vi "09_another_example.vi"() -> ()   [LabVIEW 2018, in "LV2Julia_examples.lvlib"]
uses:
  LV2Julia_examples.lvlib
  LV2Julia_core/VIs/Server or client state.ctl
  LV2Julia_core/VIs/detailed error info.ctl
  LV2Julia_core/VIs/StackFrame.ctl
  simple examples functions.ctl
  LV2Julia_core/VIs/Commands.ctl
  63b50369-e720-4ad2-b7fe-b63add1d9180.vi
  edf81fa3-46bf-427f-9605-85b461656974.vi
  29886417-d43f-41fb-9c0c-469db3f8c96d.vi
  3fe35f36-217a-40a5-a789-8326c52a1f5c.vi
  8d86b089-302c-401c-ae82-d9ebdf0ff266.vi
  35a44a82-786b-41ea-be73-9a4468e4df9d.vi
  a43e0667-dcfc-466a-94c9-f7da2d4fd36f.vi
  <vilib>/Utility/High Resolution Relative Seconds.vi
  edf81fa3-46bf-427f-9605-85b461656974.vi/5942f0bd-7063-4fdb-8e1f-163338074038.vi
  29886417-d43f-41fb-9c0c-469db3f8c96d.vi/94a9aba0-1697-4c84-91eb-fcc68cde7b35.vi
  3fe35f36-217a-40a5-a789-8326c52a1f5c.vi/ea1c78d1-8dec-492d-b19c-ac119526c4b9.vi
  35a44a82-786b-41ea-be73-9a4468e4df9d.vi/a5fe95ae-8dc8-4e69-84a5-09934be0e8db.vi
  35a44a82-786b-41ea-be73-9a4468e4df9d.vi/54b1eeee-b135-46c6-a027-240f26ec244c.vi
  35a44a82-786b-41ea-be73-9a4468e4df9d.vi/29dc6209-e462-4798-844e-48d2ff1efa69.vi
  35a44a82-786b-41ea-be73-9a4468e4df9d.vi/fb13ef7b-3dc2-43ae-b026-48829507478f.vi
  edf81fa3-46bf-427f-9605-85b461656974.vi/5942f0bd-7063-4fdb-8e1f-163338074038.vi/a212b533-a802-43cc-9280-c521d8aa8d2c.vi
  29886417-d43f-41fb-9c0c-469db3f8c96d.vi/94a9aba0-1697-4c84-91eb-fcc68cde7b35.vi/986b3ef1-05af-4579-a01d-89cf0a7e1e70.vi
  29886417-d43f-41fb-9c0c-469db3f8c96d.vi/94a9aba0-1697-4c84-91eb-fcc68cde7b35.vi/f2b0486c-a7c3-4e7a-a904-fec8be3410f0.vi
  29886417-d43f-41fb-9c0c-469db3f8c96d.vi/94a9aba0-1697-4c84-91eb-fcc68cde7b35.vi/dd0e1e63-28cb-45cd-b055-498631b7826e.vi
  3fe35f36-217a-40a5-a789-8326c52a1f5c.vi/ea1c78d1-8dec-492d-b19c-ac119526c4b9.vi/ce52c93b-e6e4-494b-9f4d-7b7b02eec5ed.vi
  3fe35f36-217a-40a5-a789-8326c52a1f5c.vi/ea1c78d1-8dec-492d-b19c-ac119526c4b9.vi/7b140ace-ff7d-49f7-89b3-e9a714b2692c.vi
  3fe35f36-217a-40a5-a789-8326c52a1f5c.vi/ea1c78d1-8dec-492d-b19c-ac119526c4b9.vi/f14f8910-dfb7-4812-9577-bccbd49d3442.vi
  35a44a82-786b-41ea-be73-9a4468e4df9d.vi/a5fe95ae-8dc8-4e69-84a5-09934be0e8db.vi/43619f87-d3a3-4430-b781-19a1ed80452b.vi
  35a44a82-786b-41ea-be73-9a4468e4df9d.vi/a5fe95ae-8dc8-4e69-84a5-09934be0e8db.vi/6bcf3c00-a23e-49d9-b22d-a7ee64d807ae.vi
  edf81fa3-46bf-427f-9605-85b461656974.vi/5942f0bd-7063-4fdb-8e1f-163338074038.vi/a212b533-a802-43cc-9280-c521d8aa8d2c.vi/2d6b78cf-7cb1-4e49-bbcd-7392787414f6.vi
  35a44a82-786b-41ea-be73-9a4468e4df9d.vi/a5fe95ae-8dc8-4e69-84a5-09934be0e8db.vi/43619f87-d3a3-4430-b781-19a1ed80452b.vi/46c53f12-cc20-4ee9-bbe7-34102a510572.vi
  LV2Julia_core/VIs/jl-scripts path.vi
  LV2Julia_core/VIs/check ID validity.vi
  LV2Julia_core/VIs/bindata_descr to JSON.vi
  LV2Julia_core/VIs/check cluster field names.vi
  LV2Julia_core/VIs/concat JSON.vi
  LV2Julia_core/VIs/build request.vi
  LV2Julia_core/VIs/Parse server response.vi
  LV2Julia_core/VIs/log jl exceptions.vi
  <vilib>/Utility/error.llb/Error Cluster From Error Code.vi
  LV2Julia_core/LV2Julia_core.lvlib
  <vilib>/measure/NI_MABase.lvlib
panel:
  out "ZMQ timeout":bool
  out "Julia script file path":path
  out "temporary script path":path
  out "Jl Server state":T1
  in  "execution control pages":enum32{"Start", "go - test"}(tab)
  in  "go":bool caption="go (Julia Server started externally)"
  in  "Start with Julia":bool caption="Start Julia Server and go"
  in  "ZMQ endpoint":string="tcp://127.0.0.1:5555"
  in  "p":dbl=1.0
  in  "fn":T2 caption="select function at Server" items=["arr_amplitude", "arr_length", "arr_mean", "arr_median", "arr_rms", "vec_amplify", "vec_attenuate", "vec_power"]
  in  "trim @ begin":dbl min=0.0 max=100.0 step=1.0 format="%#.1f%%"
  in  "trim @ end":dbl min=0.0 max=200.0 step=1.0 format="%#.1f%%"
  in  "Group":T3(tab)
  out "Server response":dbl
  out "data received plot":dbl[](graph)
  out "data received":dbl[](array[numeric]) format="%.3f"
  out "RMS":dbl
  out "detailed error info":T4
  out "current error":errorcluster
  out "final error":errorcluster
  out "short err code":u8
  in  "tones":T6(array[cluster])=[{"frequency"=10.0, "amplitude"=1.0, "phase"=0.0}, {"frequency"=20.0, "amplitude"=0.1, "phase"=0.0}] {"phase" format="%.2p"; "amplitude" format="%0.2p"; "frequency" format="%0.2p"}
  in  "noise (rms)":dbl=0.1 format="%.2p"
  in  "offset":dbl format="%.2p"
  in  "sampling info":cluster{"Fs":dbl, "#s":dbl}={"Fs"=1000.0, "#s"=1000.0} {"Fs" format="%.2p"}
  in  "next":bool
  out "data sent to server":dbl[](graph)
  out "data sent":dbl[](array[numeric]) format="%.3f"
  out "function name":string
  in  "stop this VI only":bool
  in  "stop both this VI and Julia Server":bool
  out "call duration (ms)":dbl format="%#.2f"
  # "tcp://127.0.0.1:5555 \nfor local Julia Server\n\nFor a Julia Server running on a separate computer,  you probably must use an IPv4 address in numeric form (not a DNS name) - see https://stackoverflow.com/questions/6024003/why-doesnt-zeromq-work-on-localhost.\n\nThis control only used if Julia Server is not being started by this VI."
  # "generate sample array"
  # "function and parameter"
  # "enter a negative or a large positive value to cause an exception"
  # "data returned by server"
  # "data sent to server"
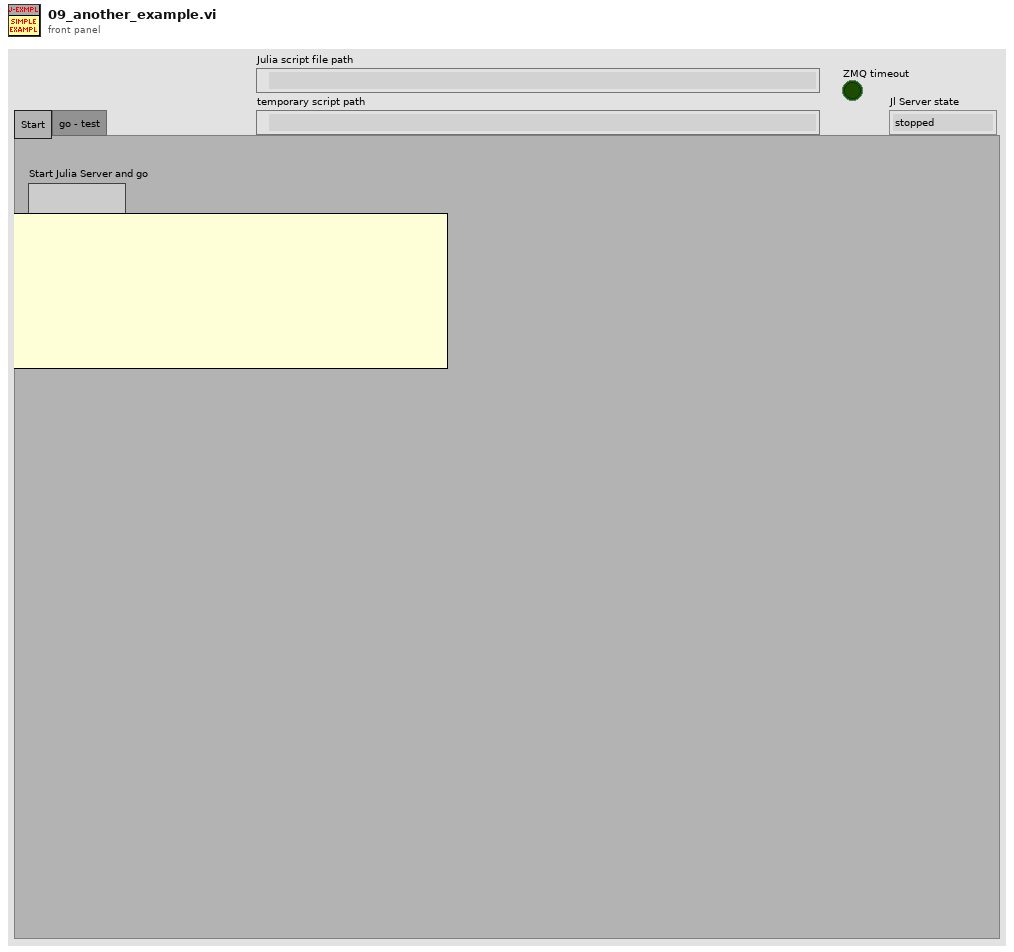
[diagram p1: front panel]
types:
  T1 = typedef "LV2Julia_core.lvlib/Server or client state.ctl" = enum16{"stopped", "running", "unknown"}
  T2 = typedef "LV2Julia_examples.lvlib/simple examples functions.ctl" = u16
  T3 = enum32{"fns returning scalar", "fns returning vector", "error"}
  T4 = typedef "LV2Julia_core.lvlib/detailed error info.ctl" = cluster{"exception_or_info":string, "trace":T5[]}
  T5 = typedef "LV2Julia_core.lvlib/StackFrame.ctl" = cluster{"frame_summary":string, "func":string, "linfo":string, "file":string, "line":i32, "pointer":u64, "from_c":bool, "inlined":bool}
  T6 = cluster{"frequency":dbl, "amplitude":dbl, "phase":dbl}[]
  T7 = typedef "LV2Julia_core.lvlib/Commands.ctl" = enum16{"Start Jl-server & Init LV-client", "Send request & Get response ", "Stop Jl-server & Cleanup LV-client", "Cleanup LV-client", "Start Jl-server", "Stop Jl-server", "Init LV-Client", "Cleanup LV-Client", "(not allowed)", "Set LV Client state", "Set Jl Server state", "set ZMQ timeout", "read ZMQ timeout", "read-out state"}
  T8 = enum8{"Enabled", "Disabled", "Disabled and Grayed Out"}
  T9 = typedef "LV2Julia_core.lvlib/Bindata&description.ctl" = cluster{"bindata_descr":T10[], "bindata":u8[]}
  T10 = typedef "LV2Julia_core.lvlib/Bindata description.ctl" = cluster{"nofbytes":i32, "numtype":string, "start":i32, "arrdims":i32[], "kwarg_name":string, "category":string}
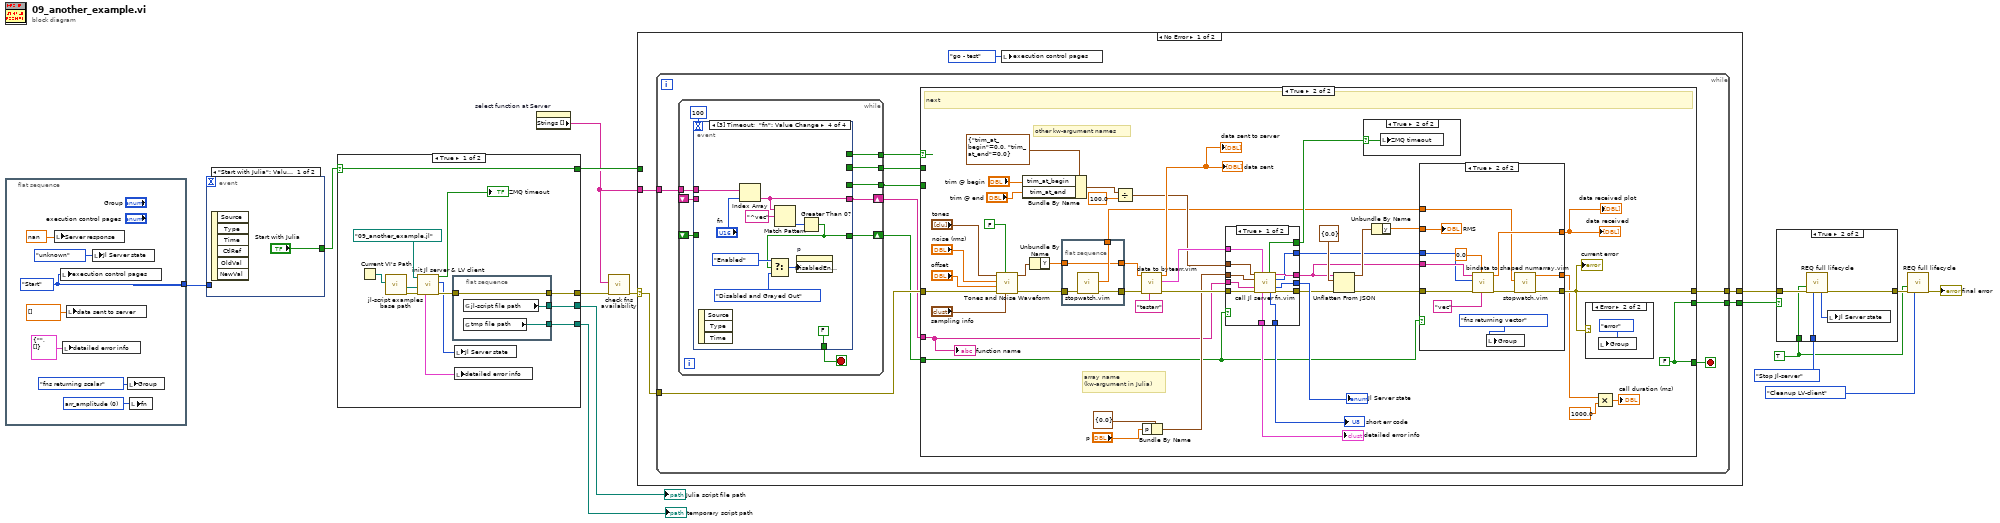
[diagram p0: block diagram]
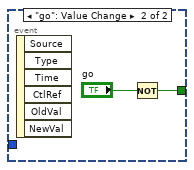
[diagram p2: hidden frame]
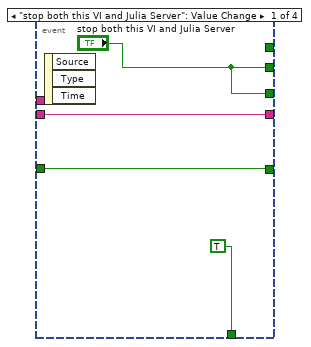
[diagram p3: hidden frame]
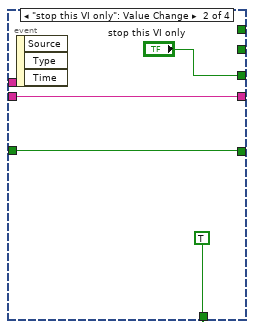
[diagram p4: hidden frame]
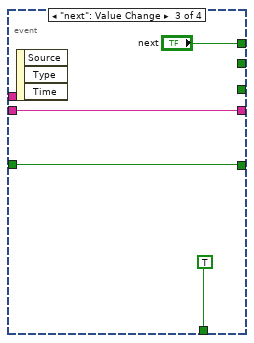
[diagram p5: hidden frame]
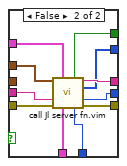
[diagram p7: hidden frame]
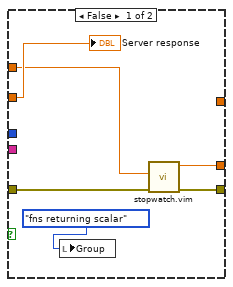
[diagram p9: hidden frame]
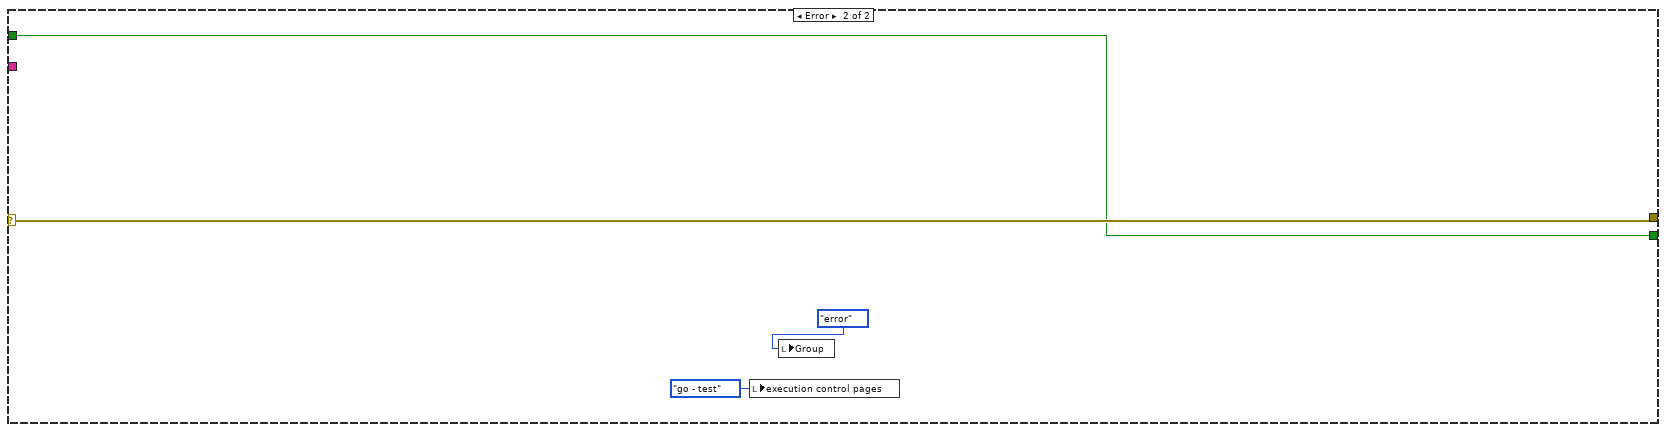
[diagram p11: hidden frame]
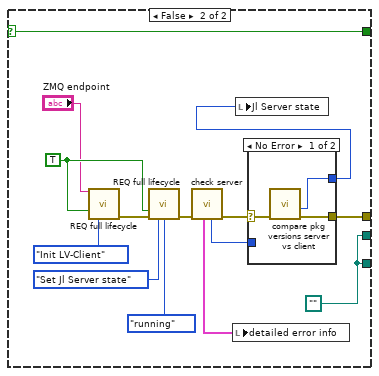
[diagram p12: hidden frame]
diagram:
  w10 = TRUE ("Force command")
  n1 = flat-sequence {
    tunnel: [w22] -> w6
    frame #0 {
      w16 = T2 0 items=["arr_amplitude", "arr_length", "arr_mean", "arr_median", "arr_rms", "vec_amplify", "vec_attenuate", "vec_power"] ("fn")
      w22 = enum32{"Start", "go - test", "finish"}."Start" ("execution control pages")
      n2 = local write "Server response"(nan ("Server response")) -> ()
      n3 = local write "execution control pages"(w22) -> ()
      n4 = local write "detailed error info"(T4 {"exception_or_info"="", "trace"=[]} ("detailed error info")) -> ()
      n5 = local write "data sent to server"(dbl[] []) -> ()
      n6 = local write "Jl Server state"(Server_or_client_state."unknown" ("Jl Server state out")) -> ()
      n7 = local write "Group"(T3."fns returning scalar" ("Group")) -> ()
      n8 = local write "fn"(w16) -> ()
    }
  }
  n9 = event shown="[0] \"Start with Julia\": Value Change" {
    selector: _ -> [_ _]
    dyn-events: _ -> [_ _]
    timeout: _ -> [_ _]
    tunnel: ["Start with Julia" w24] -> w8
    tunnel: w6 -> [_ _]
    event "Start with Julia": Value Change {
      n10 = event-data() -> ()  [unwired: 1 in, 6 out]
    }
    event "go": Value Change {
      n11 = event-data() -> ()  [unwired: 1 in, 6 out]
      n12 = Not(x="go") -> (.not. x?=w24:bool)
    }
  }
  n13 = case shown="True" w8 {
    selector: w8 -> [w37 w50]
    tunnel: [w36 w44] -> w5
    tunnel: [w37 w50] -> w7
    tunnel: [w35 w47] -> w1
    tunnel: [w34 w47] -> w2
    frame True {
      n14 = Current VI's Path() -> (path=w29:path)
      n15 = call "jl-script examples base path.vi"("calling example VI path"=w29) -> ("error out"=w28:errorcluster, "jl-script-examples base path"=w27:path)  [unwired: 9 in]
      n16 = call "init Jl server & LV client.vi"("error in (no error)"=w28, "Base path (not a path)"=w27, "Julia user functions script"=path "09_another_example.jl") -> ("error out"=w31:errorcluster, "Jl Server state out"=w30:T1, "timeout?"=→"ZMQ timeout":bool, "detailed error info"=w26:T4)  [unwired: 3 in, 2 out]
      n17 = flat-sequence {
        tunnel: [w40] -> w36
        tunnel: w31 -> [w40]
        tunnel: [w39] -> w35
        tunnel: [w38] -> w34
        frame #0 {
          n18 = global read "jl-scripts path.vi" "jl-script file path"() -> (w39:path)
          n19 = global read "jl-scripts path.vi" "tmp file path"() -> (w38:path)
        }
      }
      n20 = local write "Jl Server state"(w30) -> ()
      n21 = local write "detailed error info"(w26) -> ()
    }
    frame False {
      w47 = path ""
      w52 = TRUE ("Force command")
      n22 = call "REQ full lifecycle.vi"("ZMQ endpoint"="ZMQ endpoint", "Force command"=w52, "command"=Commands."Init LV-Client") -> ("error out"=w49:errorcluster)  [unwired: 6 in, 6 out]
      n23 = call "REQ full lifecycle.vi"("Force command"=w52, "error in"=w49, "command"=Commands."Set Jl Server state", "Jl Server state in"=Server_or_client_state."running") -> ("error out"=w48:errorcluster)  [unwired: 5 in, 6 out]
      n24 = call "check server.vi"("error in"=w48) -> ("error out"=w45:errorcluster, "Jl Server state out"=w43:T1, "detailed error info"=w41:T4)  [unwired: 6 in, 2 out]
      n25 = local write "detailed error info"(w41) -> ()
      n26 = case shown="No Error" w45 {
        selector: w45 -> [w57 w59]
        tunnel: [w56 w59] -> w44
        tunnel: [w55 w58] -> w42
        tunnel: w43 -> [_ w58]
        frame No Error {
          n27 = call "compare pkg versions server vs client.vi"("error in (no error)"=w57) -> ("error out"=w56:errorcluster, "Jl Server state out"=w55:T1)  [unwired: 5 in, 4 out]
        }
        frame Error {
        }
      }
      n28 = local write "Jl Server state"(w42) -> ()
    }
  }
  "temporary script path" <- w2
  "Julia script file path" <- w1
  n29 = property on="select function at Server" class="Ring (strict)"() -> ("Strings []"=w3:string[])  [unwired: 2 in, 2 out]
  n30 = call "check fns availability.vi"("error in (no error)"=w5, "fns list is"=w3) -> ("error out"=w4:errorcluster)  [unwired: 3 in, 6 out]
  n31 = case shown="No Error" w4 {
    selector: w4 -> [w63 w204]
    tunnel: [w64 w204] -> w15
    tunnel: [w62 w203] -> w9
    tunnel: w3 -> [w61 _]
    tunnel: w7 -> [_ w203]
    frame No Error {
      n32 = while {
        tunnel: w63 -> [w73]
        tunnel: [w74] -> w64
        tunnel: [w70] -> w62
        tunnel: w61 -> [w68]
        stop <- w71 stop-if-true
        n33 = while {
          tunnel: [w84] -> w72
          tunnel: [w83] -> w69
          tunnel: w68 -> [w80]
          shift-right: [w79] -> w67
          shift-left: _ -> [w76]
          shift-right: [w78] -> w66
          shift-left: _ -> [w77]
          tunnel: [w75] -> w65
          stop <- w82 stop-if-true
          n34 = event shown="[3] Timeout;  \"fn\": Value Change" {
            selector: _ -> [_ _ _ _]
            dyn-events: _ -> [_ _ _ _]
            timeout: 100 -> [_ _ _ _]
            tunnel: ["stop both this VI and Julia Server" _ _ _] -> w83
            tunnel: [_ _ "next" _] -> w84
            tunnel: [TRUE TRUE TRUE FALSE] -> w82
            tunnel: w80 -> [_ _ _ w100]
            tunnel: [w86 w90 w94 w99] -> w79
            tunnel: [w87 w91 w93 w98] -> w78
            tunnel: w77 -> [w87 w91 w93 _]
            tunnel: w76 -> [w86 w90 w94 _]
            tunnel: ["stop both this VI and Julia Server" "stop this VI only" _ _] -> w75
            event "stop both this VI and Julia Server": Value Change {
              n35 = event-data() -> ()  [unwired: 1 in, 3 out]
            }
            event "stop this VI only": Value Change {
              n36 = event-data() -> ()  [unwired: 1 in, 3 out]
            }
            event "next": Value Change {
              n37 = event-data() -> ()  [unwired: 1 in, 3 out]
            }
            event Timeout; Value Change {
              n38 = event-data() -> ()  [unwired: 1 in, 3 out]
              n39 = Index Array(array=w100, index="fn") -> (element=w98:string)
              n40 = Match Pattern(string=w98, regular expression="^vec") -> (offset past match=w104:i32)  [unwired: 1 in, 3 out]
              n41 = Greater Than 0?(x=w104) -> (x > 0?=w99:bool)
              n42 = Select(t=T8."Enabled" ("Disabled"), s=w99, f=T8."Disabled and Grayed Out" ("Disabled")) -> (s? t:f=w106:T8)
              n43 = property on="p" class="DigNum (strict)"("DisabledEnum"=w106) -> ()  [unwired: 2 in, 2 out]
            }
          }
        }
        n44 = case shown="True" w72 {
          tunnel: [w109 w136] -> w74
          tunnel: w73 -> [w109 w141]
          tunnel: [w108 w140] -> w71
          tunnel: w65 -> [w108 _]
          tunnel: [w107 w140] -> w70
          tunnel: w69 -> [w107 _]
          tunnel: w67 -> [_ w123]
          tunnel: w66 -> [_ w125]
          frame False {
            # "stop"
          }
          frame True {
            w140 = FALSE ("stop this VI only")
            # "other kw-argument names"
            # "array name\n(kw-argument in Julia)"
            # "next"
            n45 = call <vilib>:"Tones and Noise Waveform.vi"("sampling info"="sampling info", "reset signal"=FALSE, "error in (no error)"=w141, "offset"="offset", "noise (rms)"="noise (rms)", "tones"="tones") -> ("error out"=w115:errorcluster, "signal out"=w146:waveform(dbl))  [unwired: 4 in]
            n46 = Bundle By Name(cluster=cluster{"trim_at_begin":dbl, "trim_at_end":dbl} {"trim_at_begin"=0.0, "trim_at_end"=0.0}, "trim_at_begin"="trim @ begin", "trim_at_end"="trim @ end") -> (w120:cluster{"trim_at_begin":dbl, "trim_at_end":dbl})
            n47 = Unbundle By Name(w146) -> ("Y"=w110:dbl[])
            n48 = flat-sequence {
              tunnel: w115 -> [w157]
              tunnel: [w156] -> w114
              tunnel: [w155] -> w113
              tunnel: [w154] -> w111
              tunnel: w110 -> [w154]
              frame #0 {
                n49 = call "stopwatch.vim"("anything in"=w157) -> ("copy of anything out"=w156:errorcluster, "current timepoint"=w155:dbl)  [unwired: 8 in, 1 out]
              }
            }
            n50 = Divide(x=w120, y=100.0 ("trim @ end")) -> (x/y=w121:cluster{"trim_at_begin":dbl, "trim_at_end":dbl})
            n51 = call "data to bytearr.vim"("kwarg_name"="testarr", "error in (no error)"=w114, "data in"=w111) -> ("error out"=w134:errorcluster, "Bindata & descr out"=w127:T9, "flattened data out"=→"data sent" →"data sent to server":dbl[])  [unwired: 6 in]
            n52 = Bundle By Name(cluster=cluster{"p":dbl} {"p"=0.0}, "p"="p") -> (w126:cluster{"p":dbl})
            n53 = case shown="True" w123 {
              tunnel: w134 -> [w169 w180]
              tunnel: [w168 w179] -> w133
              tunnel: [w167 w178] -> w132
              tunnel: [w166 w177] -> w131
              tunnel: [w165 w176] -> w130
              tunnel: [w164 w175] -> w129
              tunnel: [w163 w174] -> w128
              tunnel: w127 -> [w162 w173]
              tunnel: w121 -> [w161 w172]
              tunnel: w126 -> [w160 _]
              tunnel: w125 -> [w159 w171]
              tunnel: [w158 w170] -> w124
              frame True {
                n54 = call "call Jl server fn.vim"("Arguments 1"=w161, "Bindata & descr in"=w162, "Arguments 2"=w160, "fun2call"=w159, "error in (no error)"=w169) -> ("timeout?"=w163:bool, "JSON received"=w165:string, "binary data received"=w164:u8[], "Jl Server state out"=w167:T1, "detailed error info"=w168:T4, "return code"=w158:u8, "error out"=w166:errorcluster)  [unwired: 4 in]
              }
              frame False {
                n55 = call "call Jl server fn.vim"("Arguments 1"=w172, "Bindata & descr in"=w173, "fun2call"=w171, "error in (no error)"=w180) -> ("timeout?"=w174:bool, "JSON received"=w176:string, "binary data received"=w175:u8[], "Jl Server state out"=w178:T1, "detailed error info"=w179:T4, "return code"=w170:u8, "error out"=w177:errorcluster)  [unwired: 5 in]
              }
            }
            "short err code" <- w124
            "Jl Server state" <- w132
            "detailed error info" <- w133
            n56 = Unflatten From JSON(JSON string=w130, type and defaults=cluster{"y":dbl} {"y"=0.0} ("parsed response"), error in (no error)=w131) -> (value=w152:cluster{"y":dbl}, error out=w137:errorcluster)  [unwired: 4 in]
            n57 = case shown="True" w128 {
              selector: w128 -> [_ w181]
              frame False {
              }
              frame True {
                n58 = local write "ZMQ timeout"(w181) -> ()
              }
            }
            n59 = Unbundle By Name(w152) -> ("y"=w135:dbl)
            n60 = case shown="True" w123 {
              tunnel: w137 -> [w182 w198]
              tunnel: [w183 w190] -> w136
              tunnel: w129 -> [_ w193]
              tunnel: w130 -> [_ w194]
              tunnel: w135 -> [w186 w196]
              tunnel: [w184 w188] -> w112
              tunnel: [_ w192] -> w116
              tunnel: w113 -> [w185 w189]
              frame False {
                n61 = local write "Group"(T3."fns returning scalar" ("Group")) -> ()
                n62 = call "stopwatch.vim"("anything in"=w182, "prev timepoint (0)"=w185) -> ("copy of anything out"=w183:errorcluster, "delta t (s)"=w184:dbl)  [unwired: 7 in, 1 out]
                "Server response" <- w186
              }
              frame True {
                n63 = call "bindata to shaped numarray.vim"("name"="vec" ("kwarg_name"), "element type"=0.0 ("data type"), "error in (no error)"=w198, "binary data"=w193, "JSON in"=w194) -> ("error out"=w191:errorcluster, "numarray 1D"=w192:dbl[])  [unwired: 1 in, 4 out]
                n64 = local write "Group"(T3."fns returning vector" ("Group")) -> ()
                n65 = call "stopwatch.vim"("anything in"=w191, "prev timepoint (0)"=w189) -> ("copy of anything out"=w190:errorcluster, "delta t (s)"=w188:dbl)  [unwired: 7 in, 1 out]
                "RMS" <- w196
              }
            }
            "current error" <- w136
            "data received plot" <- w116
            "data received" <- w116
            n66 = case shown="Error" w136 {
              frame No Error {
              }
              frame Error {
                n67 = local write "Group"(T3."error" ("Group")) -> ()
              }
            }
            n68 = Multiply(x=w112, y=1000.0) -> (x*y=→"call duration (ms)":dbl)
            "function name" <- w125
          }
        }
      }
      n69 = local write "execution control pages"(enum32{"Start", "go - test", "finish"}."go - test" ("execution control pages")) -> ()
    }
    frame Error {
      n70 = local write "execution control pages"(enum32{"Start", "go - test", "finish"}."go - test" ("execution control pages")) -> ()
      n71 = local write "Group"(T3."error" ("Group")) -> ()
    }
  }
  n72 = case shown="True" w9 {
    tunnel: w15 -> [w205 w210]
    tunnel: Commands."Stop Jl-server" ("command") -> [_ w209]
    tunnel: [w205 w208] -> w13
    tunnel: w10 -> [_ w207]
    frame False {
    }
    frame True {
      n73 = call "REQ full lifecycle.vi"("Force command"=w207, "error in"=w210, "command"=w209) -> ("Jl Server state out"=w206:T1, "error out"=w208:errorcluster)  [unwired: 6 in, 5 out]
      n74 = local write "Jl Server state"(w206) -> ()
    }
  }
  n75 = call "REQ full lifecycle.vi"("Force command"=w10, "error in"=w13, "command"=Commands."Cleanup LV-client") -> ("error out"=→"final error":errorcluster)  [unwired: 6 in, 6 out]
